vi "Save Report to File.vi"(0 "report in":refnum<class "ooCalc.lvclass">, 5 "report file path":path, 7 "prompt to replace? (F)":bool, 9 "password (\"\")":string, 11 "error in (no error)":errorcluster) -> (4 "report out":refnum<class "ooCalc.lvclass">, 15 "error out":errorcluster)   [LabVIEW 2009, in "ooCalc.lvclass"]
doc: "Saves an HTML report to the file specified in <B>report file path</B>. You cannot use this VI with standard reports.\n\nThis VI also saves Microsoft Word and Excel reports."
uses:
  ooCalc.lvclass
  C:/Projets/LAVAG/OpenOfficeRGT/AODL/DLLs/AODL.dll
  ooCalc.lvclass/ooCalc.ctl
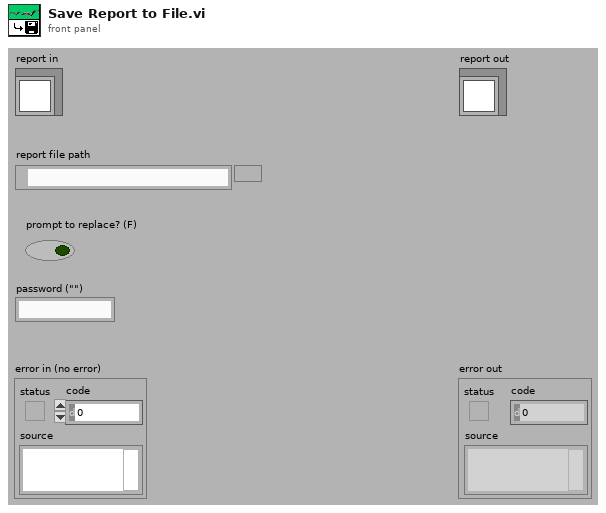
[diagram p1: front panel]
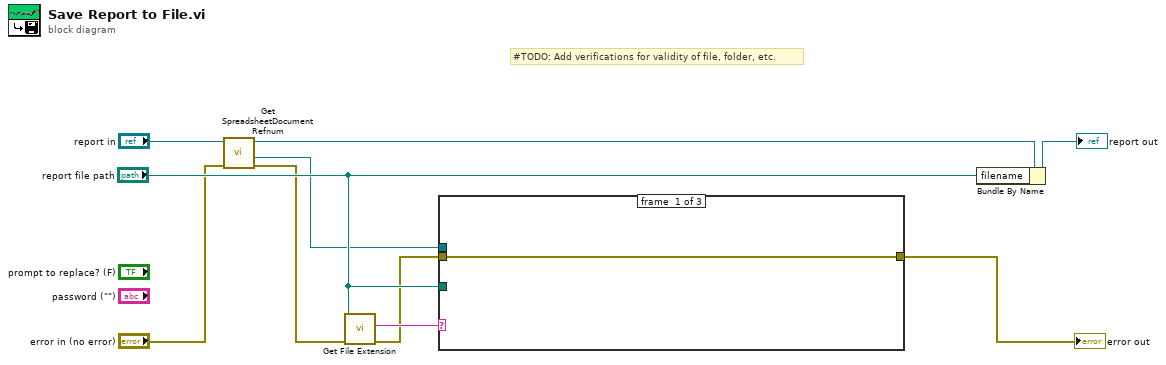
[diagram p0: block diagram]
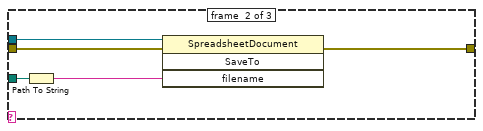
[diagram p2: hidden frame]
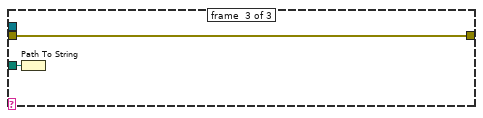
[diagram p3: hidden frame]
diagram:
  # "#TODO: Add verifications for validity of file, folder, etc."
  n1 = call-dynamic "Get SpreadsheetDocument Refnum.vi"("error in (no error)"="error in (no error)", "ooCalc in"="report in") -> ("error out"=w2:errorcluster, "SpreadsheetDocument"=w1:refnum<k24>, "ooCalc out"=w4:refnum<class "ooCalc.lvclass">)  [unwired: 7 in]
  n2 = call <vilib>:"Get File Extension.vi"("error in (no error)"=w2, "file"="report file path") -> ("error out"=w6:errorcluster, "lowercase file extension"=w8:string)  [unwired: 6 in, 2 out]
  n3 = case shown="\"ods\"" w8 {
    tunnel: w6 -> [w11 w16 w17]
    tunnel: w1 -> [_ w12 _]
    tunnel: [w11 w15 w17] -> w9
    tunnel: "report file path" -> [_ w14 w18]
    frame #0 {
    }
    frame #1 {
      n4 = Path To String(path=w14) -> (string=w13:string)
      n5 = invoke class="SpreadsheetDocument" method="SaveTo"(reference=w12, error in=w16, "filename"=w13) -> (error out=w15:errorcluster)  [unwired: 1 in, 3 out]
    }
    frame #2 {
      n6 = Path To String(path=w18) -> ()  [unwired: 1 out]
    }
  }
  "error out" <- w9
  n7 = Bundle By Name(cluster=w4, "filename"="report file path") -> (→"report out":refnum<class "ooCalc.lvclass">)
